vi "Create clusters.vi"() -> ()   [LabVIEW 2021, in "Migrator.lvlib"]
uses:
  Migrator.lvlib
panel:
  out "Cluster 2":T1
  in  "Cluster":T2
  in  "String 22":string
  out "String 21":string
  in  "Numeric 26":dbl
  in  "Numeric 25":dbl
  out "Numeric 24":dbl
  out "Numeric 23":dbl
  in  "Numeric 22":dbl
  in  "Numeric 21":dbl
  out "Numeric 20":dbl
  out "Numeric 19":dbl
  in  "Boolean 22":bool
  out "Boolean 21":bool
  in  "Boolean 20":bool
  out "Boolean 19":bool
  in  "String 20":string
  out "String 19":string
  in  "String 18":string
  out "String 17":string
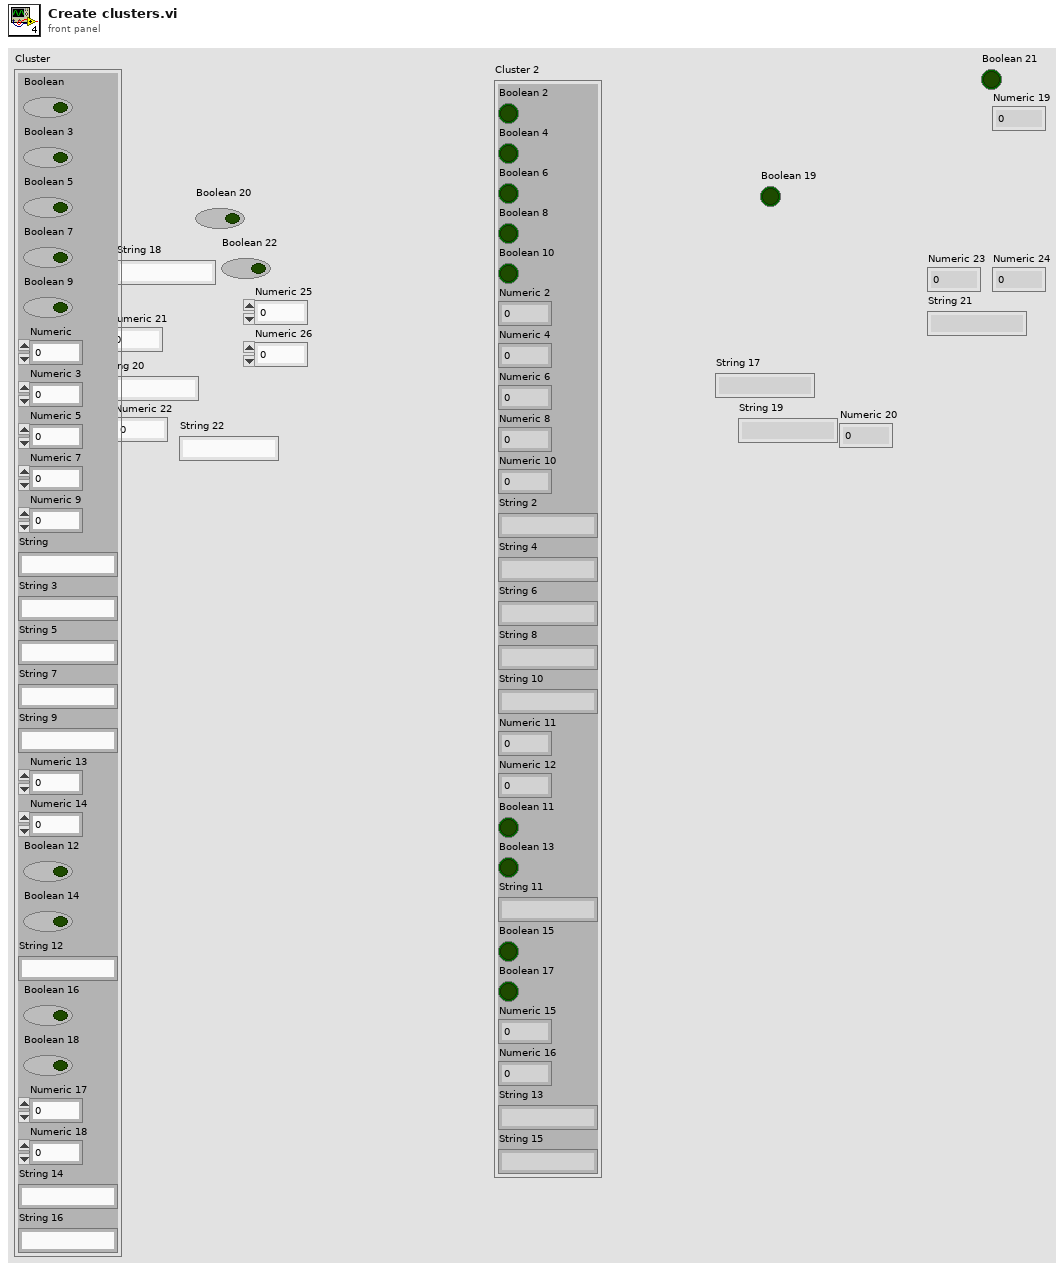
[diagram p1: front panel]
types:
  T1 = cluster{"Boolean 2":bool, "Boolean 4":bool, "Boolean 6":bool, "Boolean 8":bool, "Boolean 10":bool, "Numeric 2":dbl, "Numeric 4":dbl, "Numeric 6":dbl, "Numeric 8":dbl, "Numeric 10":dbl, "String 2":string, "String 4":string, "String 6":string, "String 8":string, "String 10":string, "Numeric 11":dbl, "Numeric 12":dbl, "Boolean 11":bool, "Boolean 13":bool, "String 11":string, "Boolean 15":bool, "Boolean 17":bool, "Numeric 15":dbl, "Numeric 16":dbl, "String 13":string, "String 15":string}
  T2 = cluster{"Boolean":bool, "Boolean 3":bool, "Boolean 5":bool, "Boolean 7":bool, "Boolean 9":bool, "Numeric":dbl, "Numeric 3":dbl, "Numeric 5":dbl, "Numeric 7":dbl, "Numeric 9":dbl, "String":string, "String 3":string, "String 5":string, "String 7":string, "String 9":string, "Numeric 13":dbl, "Numeric 14":dbl, "Boolean 12":bool, "Boolean 14":bool, "String 12":string, "Boolean 16":bool, "Boolean 18":bool, "Numeric 17":dbl, "Numeric 18":dbl, "String 14":string, "String 16":string}
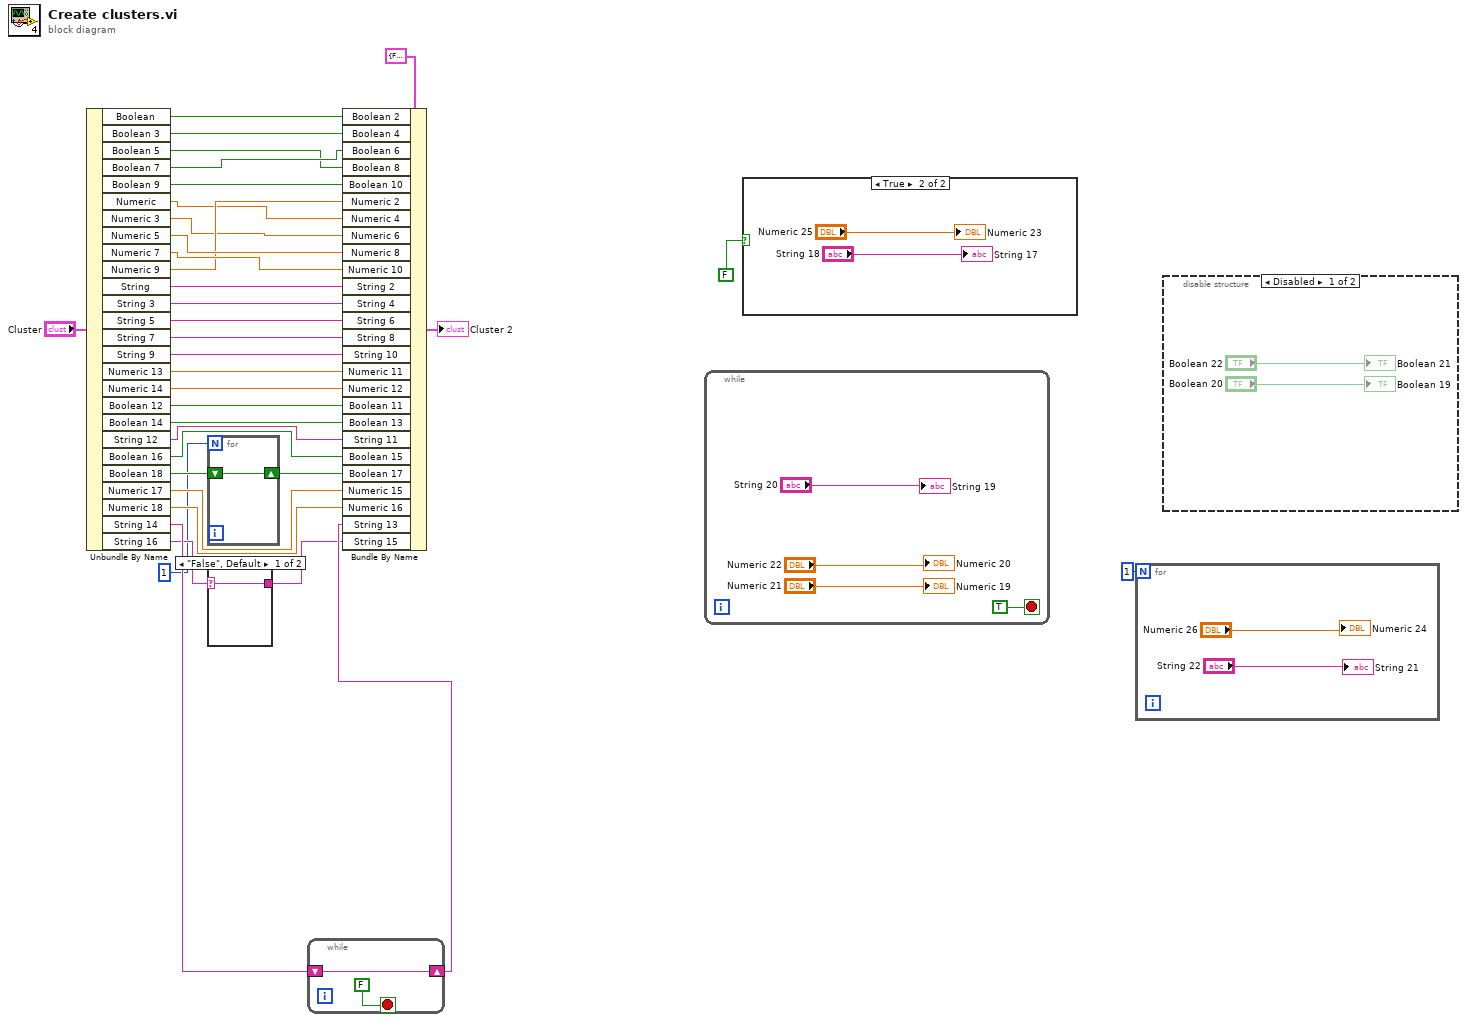
[diagram p0: block diagram]
diagram:
  n1 = Unbundle By Name("Cluster") -> ("Boolean"=w35:bool, "Boolean 3"=w34:bool, "Boolean 5"=w32:bool, "Boolean 7"=w33:bool, "Boolean 9"=w31:bool, "Numeric"=w22:dbl, "Numeric 3"=w21:dbl, "Numeric 5"=w29:dbl, "Numeric 7"=w30:dbl, "Numeric 9"=w23:dbl, "String"=w28:string, "String 3"=w27:string, "String 5"=w25:string, "String 7"=w26:string, "String 9"=w24:string, "Numeric 13"=w20:dbl, "Numeric 14"=w17:dbl, "Boolean 12"=w16:bool, "Boolean 14"=w19:bool, "String 12"=w18:string, "Boolean 16"=w15:bool, "Boolean 18"=w10:bool, "Numeric 17"=w13:dbl, "Numeric 18"=w14:dbl, "String 14"=w8:string, "String 16"=w6:string)
  n2 = for {
    N: 1 -> [_]
    shift-right: [w36] -> w9
    shift-left: w10 -> [w36]
  }
  n3 = case shown="\"False\", Default" w6 {
    selector: w6 -> [w37 w38]
    tunnel: [w37 w38] -> w5
    frame "False", Default {
    }
    frame "True" {
    }
  }
  n4 = while {
    shift-right: [w39] -> w7
    shift-left: w8 -> [w39]
    stop <- FALSE stop-if-true
  }
  n5 = Bundle By Name(cluster=T1 {"Boolean 2"=FALSE, "Boolean 4"=FALSE, "Boolean 6"=FALSE, "Boolean 8"=FALSE, "Boolean 10"=FALSE, "Numeric 2"=0.0, "Numeric 4"=0.0, "Numeric 6"=0.0, "Numeric 8"=0.0, "Numeric 10"=0.0, "String 2"="", "String 4"="", "String 6"="", "String 8"="", "String 10"="", "Numeric 11"=0.0, "Numeric 12"=0.0, "Boolean 11"=FALSE, "Boolean 13"=FALSE, "String 11"="", "Boolean 15"=FALSE, "Boolean 17"=FALSE, "Numeric 15"=0.0, "Numeric 16"=0.0, "String 13"="", "String 15"=""} ("Cluster 2"), "Boolean 2"=w35, "Boolean 4"=w34, "Boolean 6"=w33, "Boolean 8"=w32, "Boolean 10"=w31, "Numeric 2"=w23, "Numeric 4"=w22, "Numeric 6"=w21, "Numeric 8"=w29, "Numeric 10"=w30, "String 2"=w28, "String 4"=w27, "String 6"=w25, "String 8"=w26, "String 10"=w24, "Numeric 11"=w20, "Numeric 12"=w17, "Boolean 11"=w16, "Boolean 13"=w19, "String 11"=w18, "Boolean 15"=w15, "Boolean 17"=w9, "Numeric 15"=w13, "Numeric 16"=w14, "String 13"=w7, "String 15"=w5) -> (→"Cluster 2":T1)
  n6 = while {
    stop <- TRUE stop-if-true
    "Numeric 20" <- "Numeric 22"
    "Numeric 19" <- "Numeric 21"
    "String 19" <- "String 20"
  }
  n7 = case shown="True" FALSE {
    frame False {
    }
    frame True {
      "String 17" <- "String 18"
      "Numeric 23" <- "Numeric 25"
    }
  }
  n8 = for {
    N: 1 -> [_]
    "Numeric 24" <- "Numeric 26"
    "String 21" <- "String 22"
  }
  n9 = disable-structure shown="Disabled" {
    frame Disabled {
      "Boolean 21" <- "Boolean 22"
      "Boolean 19" <- "Boolean 20"
    }
    frame Enabled {
    }
  }
